vi "refresh table model.vi"(7 "engine configuration":refnum<class "engine configuration.lvclass">, 8 "error in":errorcluster, 11 "TDMS editor node":refnum<class "TDMS datalogger editor node.lvclass">) -> (0 "error out":errorcluster, 3 "TDMS editor node out":refnum<class "TDMS datalogger editor node.lvclass">, 5 "engine configuration out":refnum<class "engine configuration.lvclass">)   [LabVIEW 2015, in "TDMS datalogger editor node.lvclass"]
uses:
  TDMS datalogger editor node.lvclass
  <vilib>/NI/Module Execution Interface/Engine Configuration/engine configuration.lvclass
  <vilib>/NI/Tag Bus/tag/Data Type.ctl
  TDMS datalogger editor node.lvclass/TDMS datalogger editor node.ctl
  <vilib>/NI/Configuration Framework/serializable configuration/NISE_CEF_serializable configuration.lvclass/NISE_CEF_serializable configuration.ctl
  module/configuration/TDMS datalogger configuration.lvclass/TDMS datalogger configuration.ctl
  <vilib>/NI/Tag Bus/tag/tag descriptor.lvclass/tag descriptor.ctl
  <vilib>/NI/Module Execution Interface/Engine Configuration/engine configuration.lvclass/engine configuration.ctl
  <vilib>/NI/Tag Bus/tag/write tag name.vi
  <vilib>/NI/Tag Bus/tag/read tag name.vi
  <vilib>/NI/Tag Bus/tag/read data type.vi
  <vilib>/NI/Configuration Framework/serializable configuration/Read UID.vi
  module/configuration/Read channels.vi
  <vilib>/Utility/LVClass/Get LV Class Name.vi
  <vilib>/NI/Configuration Framework/error generator/NISE_error generator.vi
  <vilib>/NI/Tag Bus Module Framework/channel/TBM channel.lvclass
  <vilib>/NI/Tag Bus/tag/tag descriptor.lvclass
  module/configuration/TDMS datalogger configuration.lvclass
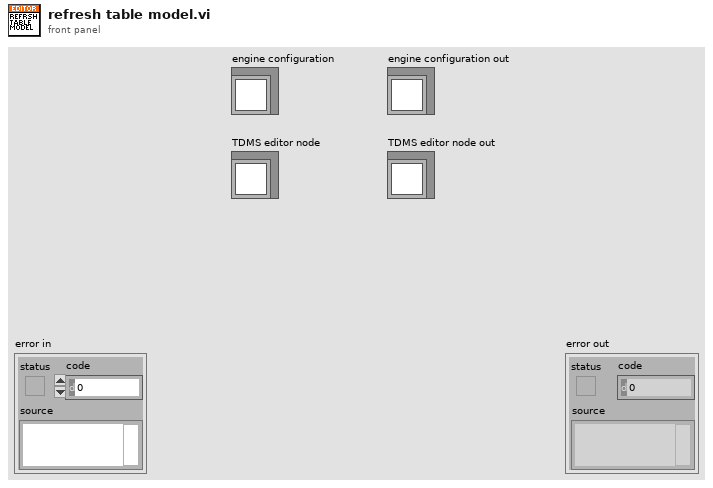
[diagram p1: front panel]
types:
  T1 = typedef "tag bus.lvlib/tag descriptor.lvclass/Data Type.ctl" = enum16{"Double", "Single", "I64", "I32", "I16", "I8", "U64", "U32", "U16", "U8", "Boolean", "String", "Array of Double", "Array of Single", "Array of I64", "Array of I32", "Array of I16", "Array of I8", "Array of U64", "Array of U32", "Array of U16", "Array of U8", "Array of Boolean", "Array of String"}
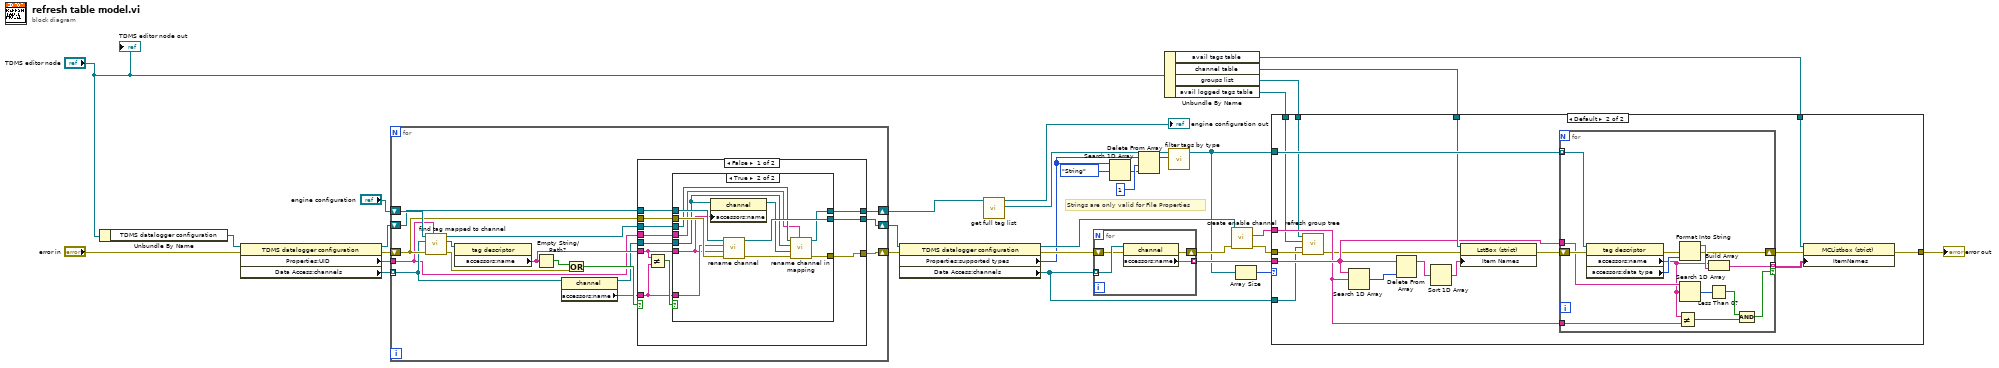
[diagram p0: block diagram]
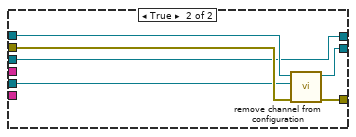
[diagram p4: hidden frame]
diagram:
  # "Strings are only valid for File Properties"
  n1 = Unbundle By Name("TDMS editor node") -> ("TDMS datalogger configuration"=w9:refnum<class "TDMS datalogger configuration.lvclass">)
  n2 = property class="TDMS datalogger configuration"(reference=w9, error in="error in") -> (reference out=w28:refnum<class "TDMS datalogger configuration.lvclass">, error out=w30:errorcluster, "Properties:UID"=w25:string, "Data Access:channels"=w31:refnum<class "TBM channel.lvclass">[])
  n3 = for {
    tunnel: w31 -> [w40] mode=indexing
    shift-right: [w35] -> w22
    shift-left: "engine configuration" -> [w48]
    shift-right: [w45] -> w27
    shift-left: w28 -> [w43]
    tunnel: w25 -> [w34]
    shift-right: [w44] -> w26
    shift-left: w30 -> [w41]
    n4 = call <vilib>:"find tag mapped to channel.vi"("owner"=w34, "error in"=w41, "channel"=w40, "engine configuration in"=w48) -> ("error out"=w39:errorcluster, "tag"=w47:refnum<class "tag descriptor.lvclass">, "engine configuration out"=w36:refnum<class "engine configuration.lvclass">)  [unwired: 5 in]
    n5 = property class="tag descriptor"(reference=w47) -> ("accessors:name"=w37:string)  [unwired: 1 in, 2 out]
    n6 = Empty String/Path?(string/path=w37) -> (empty?=w46:bool)
    n7 = property class="channel"(reference=w40) -> (reference out=w33:refnum<class "TBM channel.lvclass">, "accessors:name"=w38:string)  [unwired: 1 in, 1 out]
    n8 = Or(x=w46, y=w39) -> (x .or. y?=w42:bool)
    n9 = case shown="False" w42 {
      tunnel: [w56 w80] -> w45
      tunnel: [w59 w79] -> w44
      tunnel: w41 -> [w58 w78]
      tunnel: w43 -> [w57 w77]
      tunnel: w33 -> [w49 w76]
      tunnel: w38 -> [w54 _]
      tunnel: w37 -> [w53 _]
      tunnel: w36 -> [w52 w75]
      tunnel: [w51 w75] -> w35
      tunnel: w34 -> [w50 _]
      frame False {
        n10 = Not Equal?(x=w53, y=w54) -> (x != y?=w55:bool)
        n11 = case shown="True" w55 {
          tunnel: [w62 w67] -> w59
          tunnel: w58 -> [w62 w73]
          tunnel: w57 -> [w61 w74]
          tunnel: [w61 w72] -> w56
          tunnel: w54 -> [_ w71]
          tunnel: w53 -> [_ w64]
          tunnel: w52 -> [w60 w70]
          tunnel: [w60 w69] -> w51
          tunnel: w50 -> [_ w66]
          tunnel: w49 -> [_ w65]
          frame False {
          }
          frame True {
            n12 = property class="channel"(reference=w65, "accessors:name"=w64) -> (reference out=w63:refnum<class "TBM channel.lvclass">)  [unwired: 1 in, 1 out]
            n13 = call "rename channel.vi"("error in"=w73, "new name"=w64, "old name"=w71, "TDMS datalogger configuration in"=w74) -> ("error out"=w68:errorcluster, "TDMS datalogger configuration out"=w72:refnum<class "TDMS datalogger configuration.lvclass">)  [unwired: 6 in]
            n14 = call <vilib>:"rename channel in mapping.vi"("owner ID"=w66, "error in"=w68, "new channel"=w63, "old channel"=w65, "engine configuration in"=w70) -> ("error out"=w67:errorcluster, "engine configuration out"=w69:refnum<class "engine configuration.lvclass">)  [unwired: 5 in]
          }
        }
      }
      frame True {
        n15 = call "remove channel from configuration.vi"("error in"=w78, "TBM channel in"=w76, "TDMS datalogger configuration in"=w77) -> ("error out"=w79:errorcluster, "TDMS datalogger configuration out"=w80:refnum<class "TDMS datalogger configuration.lvclass">)  [unwired: 7 in]
      }
    }
  }
  n16 = property class="TDMS datalogger configuration"(reference=w27, error in=w26) -> (reference out=w16:refnum<class "TDMS datalogger configuration.lvclass">, error out=w24:errorcluster, "Properties:supported types"=w1:T1[], "Data Access:channels"=w13:refnum<class "TBM channel.lvclass">[])
  n17 = call <vilib>:"get full tag list.vi"("engine configuration in"=w22) -> ("tag list"=w20:refnum<class "tag descriptor.lvclass">[], "engine configuration out"=→"engine configuration out":refnum<class "engine configuration.lvclass">)  [unwired: 9 in]
  n18 = for {
    tunnel: w13 -> [w84] mode=indexing
    shift-right: [w83] -> w19
    shift-left: w24 -> [w82]
    tunnel: [w81] -> w15 mode=indexing
    n19 = property class="channel"(reference=w84, error in=w82) -> (error out=w83:errorcluster, "accessors:name"=w81:string)  [unwired: 1 out]
  }
  n20 = Search 1D Array(1D array=w1, element=Data_Type."String") -> (index of element=w2:i32)  [unwired: 1 in]
  n21 = Delete From Array(array=w1, length=1, index=w2) -> (array with subset deleted=w3:T1[])  [unwired: 1 out]
  n22 = Unbundle By Name("TDMS editor node") -> ("avail tags table"=w12:refnum<vi>, "channel table"=w11:refnum<vi>, "groups list"=w8:refnum<vi>, "avail logged tags table"=w6:refnum<vi>)
  n23 = call <vilib>:"filter tags by type.vi"("allowable types"=w3, "tags in"=w20) -> ("filtered tags"=w7:refnum<class "tag descriptor.lvclass">[])  [unwired: 9 in]
  n24 = call "create enable channel.vi"("error in"=w19, "TDMS datalogger configuration"=w16) -> ("error out"=w18:errorcluster, "enable channel name"=w17:string)  [unwired: 7 in, 1 out]
  n25 = Array Size(array=w7) -> (size(s)=w14:i32)
  n26 = case shown="Default" w14 {
    tunnel: w7 -> [_ w101]
    tunnel: [w85 w86] -> w23
    tunnel: w12 -> [_ w98]
    tunnel: w11 -> [_ w97]
    tunnel: w15 -> [_ w96]
    tunnel: w18 -> [w85 w93]
    tunnel: w17 -> [_ w95]
    tunnel: w13 -> [_ w91]
    tunnel: w8 -> [_ w90]
    tunnel: w6 -> [_ w89]
    frame 0 {
    }
    frame Default {
      n27 = call "refresh group tree.vi"("error in"=w93, "channels"=w91, "avail logged tags table"=w89, "groups list"=w90) -> ("error out"=w92:errorcluster)  [unwired: 7 in]
      n28 = Search 1D Array(1D array=w96, element=w95) -> (index of element=w102:i32)  [unwired: 1 in]
      n29 = Delete From Array(array=w96, index=w102) -> (array with subset deleted=w88:string[])  [unwired: 1 in, 1 out]
      n30 = Sort 1D Array(array=w88) -> (sorted array=w87:string[])
      n31 = property class="LstBox (strict)"(reference=w97, error in=w92, "Item Names"=w87) -> (error out=w94:errorcluster)  [unwired: 1 out]
      n32 = for {
        tunnel: w101 -> [w114] mode=indexing
        shift-right: [w111] -> w100
        shift-left: w94 -> [w113]
        tunnel: [w110] -> w99 mode=indexing if=w106
        tunnel: w96 -> [w109]
        tunnel: w95 -> [w104]
        n33 = property class="tag descriptor"(reference=w114, error in=w113) -> (error out=w112:errorcluster, "accessors:name"=w105:string, "accessors:data type"=w115:T1)  [unwired: 1 out]
        n34 = Not Equal?(x=w105, y=w104) -> (x != y?=w103:bool)
        n35 = Format Into String(error in=w112, w115) -> (resulting string=w116:string, error out=w111:errorcluster)  [unwired: 2 in]
        n36 = Search 1D Array(1D array=w109, element=w105) -> (index of element=w108:i32)  [unwired: 1 in]
        n37 = Less Than 0?(x=w108) -> (x < 0?=w107:bool)
        n38 = Build Array(w105, w116) -> (w110:string[])
        n39 = Compound Arithmetic op=AND(w107, w103) -> (w106:bool)
      }
      n40 = property class="MCListbox (strict)"(reference=w98, error in=w100, "ItemNames"=w99) -> (error out=w86:errorcluster)  [unwired: 1 out]
    }
  }
  "error out" <- w23
  "TDMS editor node out" <- "TDMS editor node"
